vi "PicoScope3000aWrap.vi"(4 "Enabled Array":i16[](array[numeric]), 5 "MSO Device?":bool, 6 "handle in":i16, 7 "error in (no error)":errorcluster) -> (0 "deviceIndex":u16, 2 "handle out":i16, 3 "error out":errorcluster)   [LabVIEW 2016]
uses:
  ps3000aWrap.dll
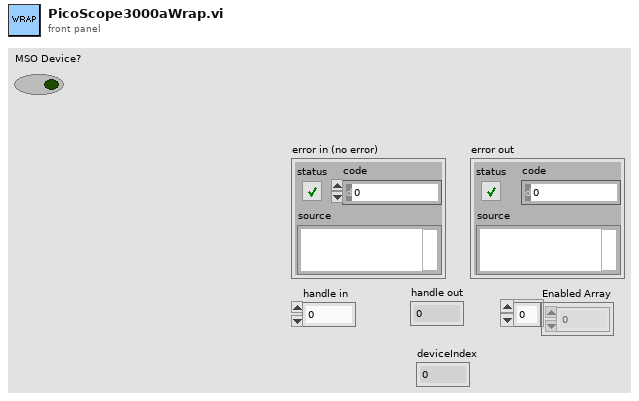
[diagram p1: front panel]
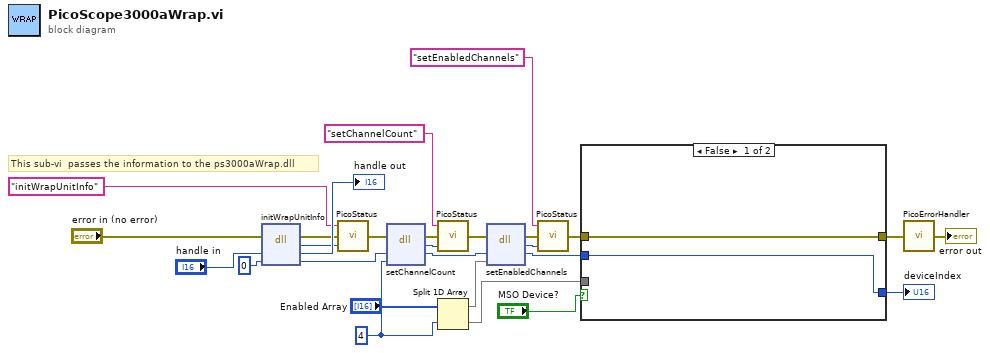
[diagram p0: block diagram]
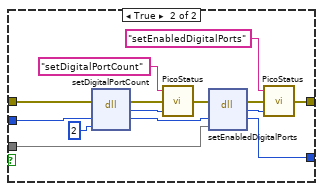
[diagram p2: hidden frame]
diagram:
  w1 = i16 4 ("channel count")
  # "This sub-vi  passes the information to the ps3000aWrap.dll"
  n1 = dll-call lib="ps3000aWrap.dll" fn="initWrapUnitInfo"(error in="error in (no error)", "handle"="handle in", "deviceIndex"=u16 0) -> (error out=w18:errorcluster, "Pico Status"=w17:u32, "handle"=→"handle out":i16, "deviceIndex"=w24:u16)  [unwired: 2 in, 1 out]
  n2 = call "PicoStatus.vi"("PICO STATUS"=w17, "error in"=w18, "source"="initWrapUnitInfo") -> ("error out"=w16:errorcluster)
  n3 = dll-call lib="ps3000aWrap.dll" fn="setChannelCount"(error in=w16, "deviceIndex"=w24, "channel count"=w1) -> (error out=w14:errorcluster, "Pico Status"=w13:u32, "deviceIndex"=w27:u16)  [unwired: 3 in, 1 out]
  n4 = call "PicoStatus.vi"("PICO STATUS"=w13, "error in"=w14, "source"="setChannelCount") -> ("error out"=w15:errorcluster)
  n5 = Split 1D Array(array="Enabled Array", index=w1) -> (first subarray=w3:i16[], second subarray=w2:i16[])
  n6 = dll-call lib="ps3000aWrap.dll" fn="setEnabledChannels"(error in=w15, "deviceIndex"=w27, "EnabledChannels"=w3) -> (error out=w12:errorcluster, "Pico Status"=w10:u32, "deviceIndex"=w21:u16)  [unwired: 3 in, 1 out]
  n7 = call "PicoStatus.vi"("PICO STATUS"=w10, "error in"=w12, "source"="setEnabledChannels") -> ("error out"=w11:errorcluster)
  n8 = case shown="False" "MSO Device?" {
    tunnel: w11 -> [w29 w43]
    tunnel: [w29 w35] -> w5
    tunnel: w21 -> [w28 w42]
    tunnel: [w28 w39] -> w20
    tunnel: w2 -> [_ w30]
    frame False {
    }
    frame True {
      n9 = dll-call lib="ps3000aWrap.dll" fn="setDigitalPortCount"(error in=w43, "deviceIndex"=w42, "DigitalPortCount"=i16 2) -> (error out=w38:errorcluster, "Pico Status"=w37:u32, "deviceIndex"=w40:u16)  [unwired: 3 in, 1 out]
      n10 = call "PicoStatus.vi"("PICO STATUS"=w37, "error in"=w38, "source"="setDigitalPortCount") -> ("error out"=w33:errorcluster)
      n11 = dll-call lib="ps3000aWrap.dll" fn="setEnabledDigitalPorts"(error in=w33, "deviceIndex"=w40, "EnabledDigitalChannels"=w30) -> (error out=w36:errorcluster, "Pico Status"=w34:u32, "deviceIndex"=w39:u16)  [unwired: 3 in, 1 out]
      n12 = call "PicoStatus.vi"("PICO STATUS"=w34, "error in"=w36, "source"="setEnabledDigitalPorts") -> ("error out"=w35:errorcluster)
    }
  }
  "deviceIndex" <- w20
  n13 = call "PicoErrorHandler.vi"("error in"=w5) -> ("error out"=→"error out":errorcluster)
